vi "PicoScope2000FrequencyToDeltaPhase.vi"(2 "size":i32, 3 "frequency":dbl) -> (0 "deltaPhase":dbl)   [LabVIEW 2009]
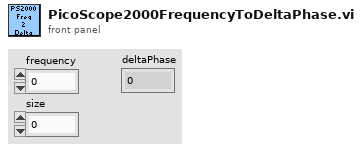
[diagram p1: front panel]
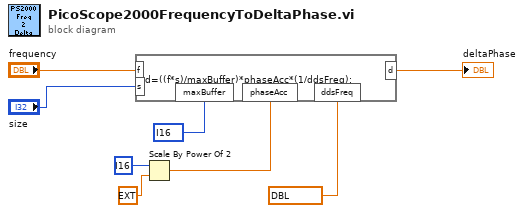
[diagram p0: block diagram]
diagram:
  n1 = Scale By Power Of 2(n=i16 ?, x=ext ?) -> (x*2^n=w6:ext)
  n2 = formula code="d=((f*s)/maxBuffer)*phaseAcc*(1/ddsFreq);"("f"="frequency", "s"="size", "phaseAcc"=w6, "maxBuffer"=i16 ? ("input variable"), "ddsFreq"=dbl ? ("input variable")) -> ("d"=→"deltaPhase":dbl)
